vi "GetClientComplexityv1.vi"() -> ()   [LabVIEW 2017]
uses:
  <userlib>/_RADE/japc/classes/JGet/JGet.lvclass
panel:
  out "error out":errorcluster
  out "test_property":T1
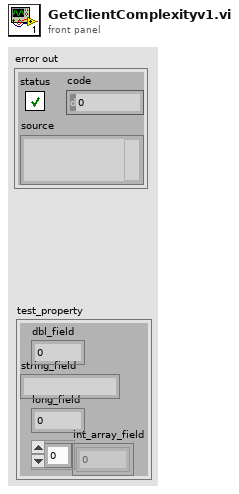
[diagram p1: front panel]
types:
  T1 = cluster{"dbl_field":dbl, "string_field":string, "long_field":i64, "int_array_field":i32[]}
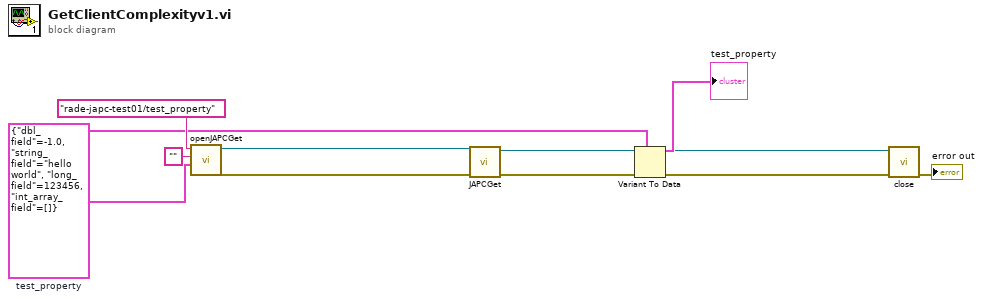
[diagram p0: block diagram]
diagram:
  w8 = T1 {"dbl_field"=-1.0, "string_field"="hello world", "long_field"=123456, "int_array_field"=[]}  # test_property
  n1 = call <userlib>:"openJAPCGet.vi"("Data type"=w8, "Cycle"="", "URL"="rade-japc-test01/test_property") -> ("error out"=w1:errorcluster, "Object out"=w4:refnum<class "JGet.lvclass">)  [unwired: 7 in]
  n2 = call <userlib>:"JAPCGet.vi"("error in (no error)"=w1, "Object in"=w4) -> ("error out"=w2:errorcluster, "Object out"=w3:refnum<class "JGet.lvclass">)  [unwired: 5 in, 3 out]
  n3 = Variant To Data(error in=w2, type=w8) -> (data=→"test_property":T1, error out=w6:errorcluster)  [unwired: 1 in]
  n4 = call-dynamic "close.vi"("error in (no error)"=w6, "Object in"=w3) -> ("error out"=→"error out":errorcluster)  [unwired: 9 in]
